vi "libssh2_agent_init.vi"(8 "error in (no error)":errorcluster, 11 "session":T1) -> (0 "error out":errorcluster, 3 "agent":T2)   [LabVIEW 2017, in "libssh2.lvlib"]
doc: "Initialize an SSH agent handle. The caller is responsible for releasing the handle by calling <B>libssh2_agent_free</B>."
uses:
  libssh2.lvlib
  Agent Refnum.ctl
  Session Refnum.ctl
  Not A Session.vi
  <vilib>/Utility/error.llb/Error Cluster From Error Code.vi
  Global Settings.vi
  Read Session Refnum.vi
  <vilib>/Utility/semaphor.llb/Acquire Semaphore.vi
  <vilib>/Utility/semaphor.llb/Release Semaphore.vi
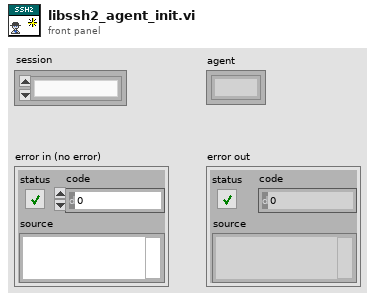
[diagram p1: front panel]
types:
  T1 = typedef "libssh2.lvlib/Session Refnum.ctl" = refnum<k1>
  T2 = typedef "libssh2.lvlib/Agent Refnum.ctl" = refnum<k1>
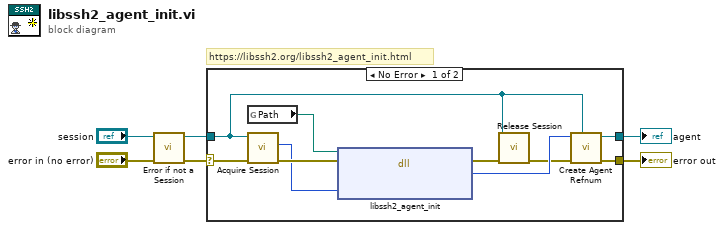
[diagram p0: block diagram]
diagram:
  # "https://libssh2.org/libssh2_agent_init.html"
  n1 = call "Error if not a Session.vi"("error in (no error)"="error in (no error)", "session"="session") -> ("error out"=w3:errorcluster, "session out"=w2:T1)  [unwired: 8 in]
  n2 = case shown="No Error" w3 {
    selector: w3 -> [w14 w17]
    tunnel: [w16 _] -> w4
    tunnel: [w15 w17] -> w6
    tunnel: w2 -> [w7 _]
    frame No Error {
      n3 = global read "Global Settings.vi" "Path"() -> (w11:path)
      n4 = call "Acquire Session.vi"("error in (no error)"=w14, "session"=w7) -> ("error out"=w10:errorcluster, "LIBSSH2_SESSION*"=w9:u64)  [unwired: 7 in, 1 out]
      n5 = dll-call lib="?" fn="libssh2_agent_init"(path in=w11, error in=w10, "session"=w9) -> (error out=w12:errorcluster, "return value"=w13:u64)  [unwired: 2 in, 1 out]
      n6 = call "Release Session.vi"("error in (no error)"=w12, "session"=w7) -> ("error out"=w8:errorcluster)  [unwired: 9 in]
      n7 = call "Create Agent Refnum.vi"("session"=w7, "error in (no error)"=w8, "LIBSSH2_AGENT*"=w13) -> ("error out"=w15:errorcluster, "agent"=w16:T2)  [unwired: 7 in]
    }
    frame Error {
    }
  }
  "error out" <- w6
  "agent" <- w4
